vi "Inspect_Width.vi"(9 "Width Tol (mm)":dbl, 10 "Nominal Width (mm)":dbl, 11 "Image":u8[][](array[numeric])) -> (1 "Width OK":bool, 2 "Width Defect":string, 3 "Width (mm)":dbl)   [LabVIEW 2018]
doc: "Use this template to build a VI to use as a subVI."
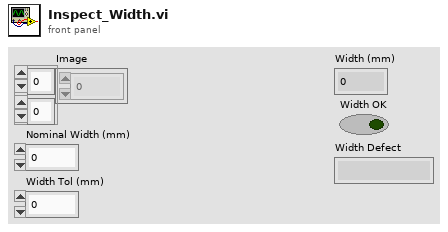
[diagram p1: front panel]
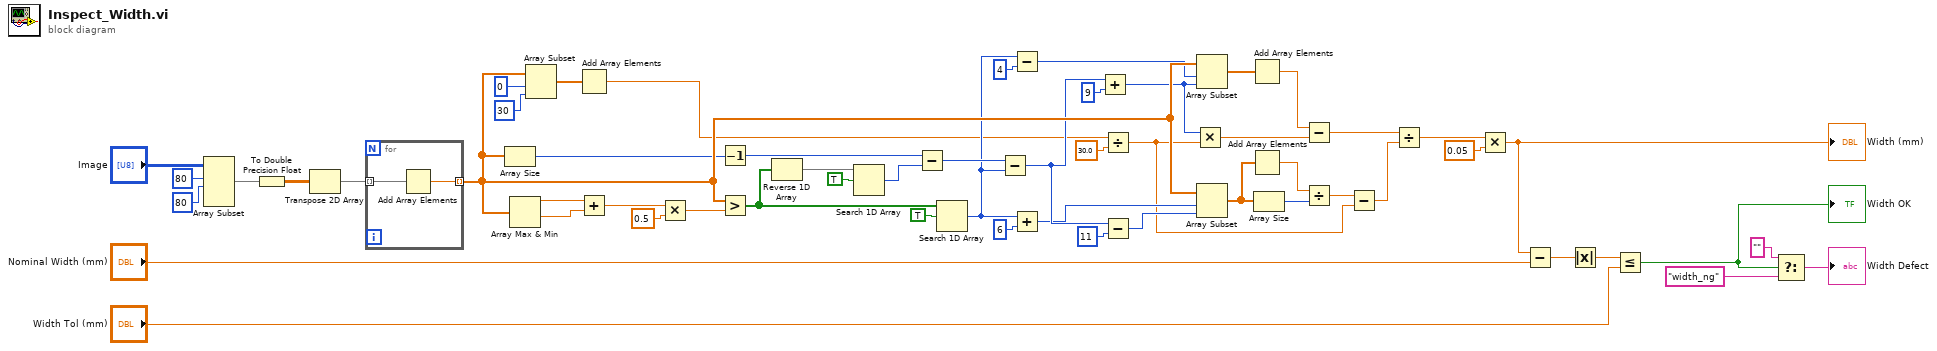
[diagram p0: block diagram]
diagram:
  n1 = Array Subset(array="Image", index (row)=80 ("index"), length (row)=80 ("length")) -> (w53:u8[][])  [unwired: 2 in]
  n2 = To Double Precision Float(number=w53) -> (double precision float=w52:dbl[][])
  n3 = Transpose 2D Array(2D array=w52) -> (transposed array=w51:dbl[][])
  n4 = for {
    tunnel: w51 -> [w58] mode=indexing
    tunnel: [w57] -> w50 mode=indexing
    n5 = Add Array Elements(numeric array=w58) -> (sum=w57:dbl)
  }
  n6 = Array Size(array=w50) -> (size(s)=w40:i32)
  n7 = Array Max & Min(array=w50) -> (max value=w49:dbl, min value=w48:dbl)  [unwired: 2 out]
  n8 = Array Subset(array=w50, index=0, length=30) -> (w27:dbl[])
  n9 = Add Array Elements(numeric array=w27) -> (sum=w26:dbl)
  n10 = Add(x=w49, y=w48) -> (x+y=w47:dbl)
  n11 = Multiply(x=w47, y=0.5) -> (x*y=w45:dbl)
  n12 = Decrement(x=w40) -> (x-1=w39:i32)
  n13 = Greater?(x=w50, y=w45) -> (0:w44:bool[])
  n14 = Reverse 1D Array(array=w44) -> (reversed array=w42:bool[])
  n15 = Search 1D Array(1D array=w42, element=TRUE) -> (index of element=w38:i32)  [unwired: 1 in]
  n16 = Subtract(x=w39, y=w38) -> (x-y=w37:i32)
  n17 = Search 1D Array(1D array=w44, element=TRUE) -> (index of element=w36:i32)  [unwired: 1 in]
  n18 = Subtract(x=w37, y=w36) -> (x-y=w35:i32)
  n19 = Subtract(x=w36, y=4) -> (x-y=w32:i32)
  n20 = Add(x=w36, y=6) -> (x+y=w22:i32)
  n21 = Add(x=w35, y=9) -> (x+y=w31:i32)
  n22 = Divide(x=w26, y=30.0) -> (x/y=w17:dbl)
  n23 = Subtract(x=w35, y=11) -> (x-y=w21:i32)
  n24 = Multiply(x=w31, y=w17) -> (x*y=w15:dbl)
  n25 = Array Subset(array=w50, index=w32, length=w31) -> (w30:dbl[])
  n26 = Array Subset(array=w50, index=w22, length=w21) -> (w20:dbl[])
  n27 = Add Array Elements(numeric array=w30) -> (sum=w16:dbl)
  n28 = Add Array Elements(numeric array=w20) -> (sum=w19:dbl)
  n29 = Array Size(array=w20) -> (size(s)=w18:i32)
  n30 = Subtract(x=w16, y=w15) -> (x-y=w13:dbl)
  n31 = Divide(x=w19, y=w18) -> (x/y=w14:dbl)
  n32 = Subtract(x=w14, y=w17) -> (x-y=w12:dbl)
  n33 = Divide(x=w13, y=w12) -> (x/y=w11:dbl)
  n34 = Multiply(x=w11, y=0.05) -> (x*y=w9:dbl)
  "Width (mm)" <- w9
  n35 = Subtract(x=w9, y="Nominal Width (mm)") -> (x-y=w7:dbl)
  n36 = Absolute Value(x=w7) -> (abs(x)=w6:dbl)
  n37 = Less Or Equal?(x=w6, y="Width Tol (mm)") -> (x <= y?=w4:bool)
  "Width OK" <- w4
  n38 = Select(t="", s=w4, f="width_ng") -> (s? t:f=→"Width Defect":string)
